vi "measure SEM Measurement.vi"(8 "error in (no error)":errorcluster, 9 "RU":i32, 10 "Center Frequency":dbl, 11 "SA Measurement in":refnum<class "SA Measurement.lvclass">) -> (0 "error out":errorcluster, 2 "Pass?":bool, 3 "SA Measurement out":refnum<class "SA Measurement.lvclass">)   [LabVIEW 2023, in "Spectrum Analyzer.lvlib" / "SA Measurement.lvclass"]
uses:
  SA Measurement.lvclass
  SA Measurement.lvclass/SA Measurement.ctl
  TYPE DEFINITION/Keysight 9020A/TYPE Measurement Preset.ctl
  Spectrum Analyzer.lvlib
  TYPE DEFINITION/TYPE RBW and VBW Select.ctl
  Interface_Spectrum/Interface_Spectrum.lvclass
  TYPE DEFINITION/TYPE Marker Peak Search Type.ctl
  TYPE DEFINITION/TYPE Limit Line Setting Table.ctl
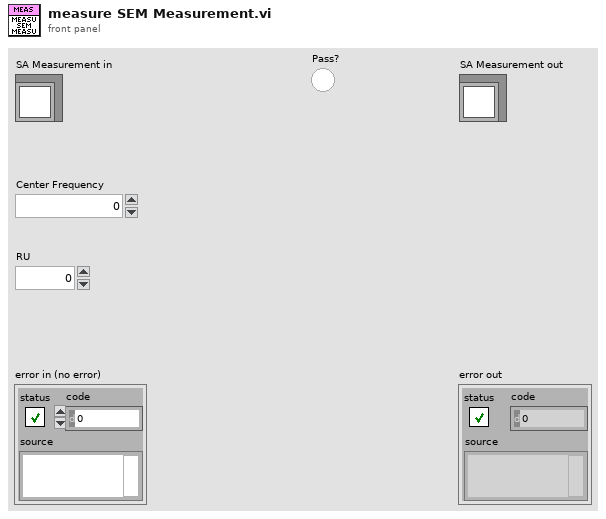
[diagram p1: front panel]
types:
  T1 = typedef "Spectrum Analyzer.lvlib/TYPE Marker Peak Search Type.ctl" = enum16{"Max", "Next Peak"}
  T2 = typedef "Spectrum Analyzer.lvlib/TYPE Limit Line Setting Table.ctl" = cluster{"Limit Line Index":i32, "Frequency Table":dbl[], "Amplitude Table":dbl[], "Name":string}
  T3 = typedef "Spectrum Analyzer.lvlib/TYPE RBW and VBW Select.ctl" = enum16{"Res BW", "Video BW"}
  T4 = typedef "Spectrum Analyzer.lvlib/TYPE Measurement Preset.ctl" = enum16{"Sweep SA Mode", "Channel Power", "Occupied BW", "ACP", "Spurious Emission", "Spurious Emission Mask", "Burst Power (Transmit Power)"}
  T5 = typedef "Spectrum Analyzer.lvlib/TYPE Mask Table for SEM.ctl" = map{enum16{"-10dBm Upper", "-10dBm Lower"}, map{dbl, map{i32, cluster{"Freq":dbl, "Limit":dbl, "dBc Applied?":bool}[]}}}
  T6 = typedef "Spectrum Analyzer.lvlib/TYPE Y-axis Unit.ctl" = enum16{"dBm", "dBmV", "dBuV", "dBpW", "Volt", "Ampere", "Watt"}
  T7 = typedef "Spectrum Analyzer.lvlib/TYPE Reference Level and Atten Param.ctl" = cluster{"Reference Level":dbl, "Atten":i32, "Atten Auto?":bool, "Reference Level Offset":dbl}
  T8 = typedef "Spectrum Analyzer.lvlib/TYPE Start and Stop Frequency.ctl" = cluster{"Start":dbl, "Stop":dbl}
  T9 = typedef "Spectrum Analyzer.lvlib/TYPE Display Trace Mode Select.ctl" = enum16{"Clear Write", "Max Hold", "Min Hold", "Average", "View"}
  T10 = typedef "Spectrum Analyzer.lvlib/TYPE Detect Mode Select.ctl" = enum16{"Det Auto (Normal)", "Auto Peak", "Positive Peak", "Negative Peak", "Sample", "RMS", "Average", "Quasipeak", "CISPR Average", "RMS Average"}
  T11 = cluster{"Trace Mode":T9, "Detector Type":T10, "Detect Auto?":bool}[]
  T12 = typedef "Spectrum Analyzer.lvlib/TYPE Average Mode Select.ctl" = enum16{"Linear(Voltage Avg)", "Video(Log)", "Power"}
  T13 = typedef "Spectrum Analyzer.lvlib/TYPE Marker Value.ctl" = cluster{"X-axis":dbl, "Y-axis":dbl}
  T14 = map{dbl, map{i32, cluster{"Freq":dbl, "Limit":dbl, "dBc Applied?":bool}[]}}
  T15 = map{i32, cluster{"Freq":dbl, "Limit":dbl, "dBc Applied?":bool}[]}
  T16 = cluster{"Freq":dbl, "Limit":dbl, "dBc Applied?":bool}[]
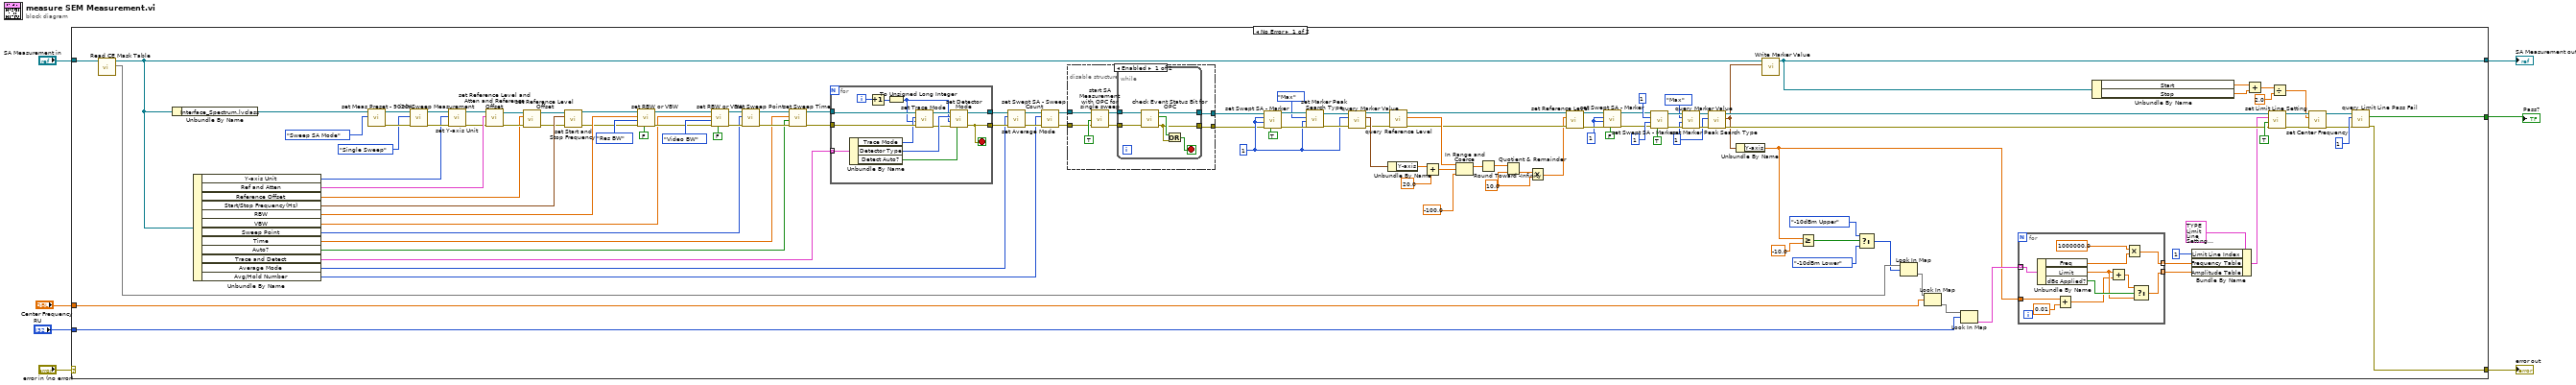
[diagram p0: block diagram]
diagram:
  n1 = case shown="No Error" "error in (no error)" {
    selector: "error in (no error)" -> [_ w167]
    tunnel: [w89 w167] -> w4
    tunnel: [w39 w166] -> w5
    tunnel: "SA Measurement in" -> [w68 w166]
    tunnel: [w88 _] -> w3
    tunnel: "Center Frequency" -> [w66 _]
    tunnel: "RU" -> [w65 _]
    frame No Error {
      w9 = 10.0 ("y")
      w16 = 1 ("Index")
      w31 = 1 ("Index")
      w71 = 1 ("Marker Index")
      n2 = call "Read CE Mask Table.vi"("SA Measurement in"=w68) -> ("Mask Table"=w55:T5, "SA Measurement out"=w41:refnum<class "SA Measurement.lvclass">)  [unwired: 8 in, 1 out]
      n3 = Unbundle By Name(w41) -> ("Interface_Spectrum.lvclass"=w127:refnum<class "Interface_Spectrum.lvclass">)
      n4 = Unbundle By Name(w41) -> ("Y-axis Unit"=w109:T6, "Ref and Atten"=w122:T7, "Reference Offset"=w80:dbl, "Start/Stop Frequency(Hz)"=w92:T8, "RBW"=w121:dbl, "VBW"=w114:dbl, "Sweep Point"=w106:u32, "Time"=w103:dbl, "Auto?"=w102:bool, "Trace and Detect"=w99:T11, "Average Mode"=w96:T12, "Avg/Hold Number"=w93:u32)
      n5 = call-dynamic "set Meas Preset - 9020A.vi"("Measurement Preset"=TYPE_Measurement_Preset."Sweep SA Mode", "Interface_Spectrum in"=w127) -> ("error out"=w124:errorcluster, "Interface_Spectrum out"=w125:refnum<class "Interface_Spectrum.lvclass">)  [unwired: 8 in]
      n6 = call-dynamic "init Sweep Measurement.vi"("error in (no error)"=w124, "Sweep Measurement Mode"=enum16{"Single Sweep", "Continuous Sweep"}."Single Sweep", "Interface_Spectrum in"=w125) -> ("error out"=w112:errorcluster, "Interface_Spectrum out"=w113:refnum<class "Interface_Spectrum.lvclass">)  [unwired: 7 in]
      n7 = call-dynamic "set Y-axis Unit.vi"("error in (no error)"=w112, "Y-axis Unit"=w109, "Interface_Spectrum in"=w113) -> ("error out"=w110:errorcluster, "Interface_Spectrum out"=w111:refnum<class "Interface_Spectrum.lvclass">)  [unwired: 7 in]
      n8 = call-dynamic "set Reference Level and Atten and Reference Offset.vi"("error in (no error)"=w110, "Reference Level, Atten, Reference Offset"=w122, "Interface_Spectrum in"=w111) -> ("error out"=w83:errorcluster, "Interface_Spectrum out"=w84:refnum<class "Interface_Spectrum.lvclass">)  [unwired: 7 in]
      n9 = call-dynamic "set Reference Level Offset.vi"("error in (no error)"=w83, "Reference Level Offset"=w80, "Interface_Spectrum in"=w84) -> ("error out"=w81:errorcluster, "Interface_Spectrum out"=w82:refnum<class "Interface_Spectrum.lvclass">)  [unwired: 7 in]
      n10 = call-dynamic "set Start and Stop Frequency.vi"("error in (no error)"=w81, "Start/Stop Frequency(Hz)"=w92, "Interface_Spectrum in"=w82) -> ("error out"=w90:errorcluster, "Interface_Spectrum out"=w91:refnum<class "Interface_Spectrum.lvclass">)  [unwired: 7 in]
      n11 = call-dynamic "set RBW or VBW.vi"("BW Auto?"=FALSE, "error in (no error)"=w90, "BW Type"=TYPE_RBW_and_VBW_Select."Res BW", "BW Value (Hz)"=w121, "Interface_Spectrum in"=w91) -> ("error out"=w115:errorcluster, "Interface_Spectrum out"=w116:refnum<class "Interface_Spectrum.lvclass">)  [unwired: 5 in]
      n12 = call-dynamic "set RBW or VBW.vi"("BW Auto?"=FALSE, "error in (no error)"=w115, "BW Type"=TYPE_RBW_and_VBW_Select."Video BW", "BW Value (Hz)"=w114, "Interface_Spectrum in"=w116) -> ("error out"=w107:errorcluster, "Interface_Spectrum out"=w108:refnum<class "Interface_Spectrum.lvclass">)  [unwired: 5 in]
      n13 = call-dynamic "set Sweep Point.vi"("error in (no error)"=w107, "Sweep Point"=w106, "Interface_Spectrum in"=w108) -> ("error out"=w104:errorcluster, "Interface_Spectrum out"=w105:refnum<class "Interface_Spectrum.lvclass">)  [unwired: 7 in]
      n14 = call-dynamic "set Sweep Time.vi"("error in (no error)"=w104, "Sweep Time Auto?"=w102, "Sweep Time(sec)"=w103, "Interface_Spectrum in"=w105) -> ("error out"=w100:errorcluster, "Interface_Spectrum out"=w101:refnum<class "Interface_Spectrum.lvclass">)  [unwired: 6 in]
      n15 = for {
        tunnel: w101 -> [w164]
        tunnel: w100 -> [w163]
        tunnel: w99 -> [w165] mode=indexing
        tunnel: [w153] -> w97
        tunnel: [w154] -> w98
        i -> [w162]
        stop <- w153 stop-if-true
        n16 = Unbundle By Name(w165) -> ("Trace Mode"=w160:T9, "Detector Type"=w158:T10, "Detect Auto?"=w155:bool)
        n17 = Increment(x=w162) -> (x+1=w161:i32)
        n18 = To Unsigned Long Integer(number=w161) -> (unsigned 32bit integer=w156:u32)
        n19 = call-dynamic "set Trace Mode.vi"("error in (no error)"=w163, "Trace Index"=w156, "Trace Mode"=w160, "Interface_Spectrum in"=w164) -> ("error out"=w157:errorcluster, "Interface_Spectrum out"=w159:refnum<class "Interface_Spectrum.lvclass">)  [unwired: 6 in]
        n20 = call-dynamic "set Detector Mode.vi"("Detect Auto?"=w155, "error in (no error)"=w157, "Trace Index"=w156, "Detector Type"=w158, "Interface_Spectrum in"=w159) -> ("error out"=w153:errorcluster, "Interface_Spectrum out"=w154:refnum<class "Interface_Spectrum.lvclass">)  [unwired: 5 in]
      }
      n21 = call-dynamic "set Average Mode.vi"("error in (no error)"=w97, "Average Mode"=w96, "Interface_Spectrum in"=w98) -> ("error out"=w94:errorcluster, "Interface_Spectrum out"=w95:refnum<class "Interface_Spectrum.lvclass">)  [unwired: 7 in]
      n22 = call-dynamic "set Swept SA - Sweep Count.vi"("error in (no error)"=w94, "Sweep Count"=w93, "Interface_Spectrum in"=w95) -> ("error out"=w85:errorcluster, "Interface_Spectrum out"=w86:refnum<class "Interface_Spectrum.lvclass">)  [unwired: 7 in]
      n23 = disable-structure shown="Enabled" {
        disable-tunnel: [w142 w152] -> w15
        disable-tunnel: [w141 _] -> w14
        disable-tunnel: w86 -> [w140 w152]
        disable-tunnel: w85 -> [w139 _]
        frame Enabled {
          n24 = call-dynamic "start SA Measurement with OPC for single sweep.vi"("error in (no error)"=w139, "with OPC?"=TRUE, "Interface_Spectrum in"=w140) -> ("error out"=w143:errorcluster, "Interface_Spectrum out"=w144:refnum<class "Interface_Spectrum.lvclass">)  [unwired: 7 in]
          n25 = while {
            tunnel: w144 -> [w151]
            tunnel: w143 -> [w150]
            tunnel: [w147] -> w141
            tunnel: [w146] -> w142
            stop <- w148 stop-if-true
            n26 = call-dynamic "check Event Status Bit for OPC.vi"("error in (no error)"=w150, "Interface_Spectrum in"=w151) -> ("error out"=w147:errorcluster, "OPC Bit Changed?"=w149:bool, "Interface_Spectrum out"=w146:refnum<class "Interface_Spectrum.lvclass">)  [unwired: 7 in]
            n27 = Or(x=w149, y=w147) -> (x .or. y?=w148:bool)
          }
        }
        frame Disabled {
        }
      }
      n28 = call-dynamic "set Swept SA - Marker.vi"("On?"=TRUE, "error in (no error)"=w14, "trace"=w31, "Index"=w31, "Interface_Spectrum in"=w15) -> ("error out"=w35:errorcluster, "Interface_Spectrum out"=w36:refnum<class "Interface_Spectrum.lvclass">)  [unwired: 5 in]
      n29 = call-dynamic "set Marker Peak Search Type.vi"("error in (no error)"=w35, "Marker Index"=w31, "Peak Search Type"=TYPE_Marker_Peak_Search_Type."Max", "Interface_Spectrum in"=w36) -> ("error out"=w32:errorcluster, "Interface_Spectrum out"=w33:refnum<class "Interface_Spectrum.lvclass">)  [unwired: 6 in]
      n30 = call-dynamic "query Marker Value.vi"("error in (no error)"=w32, "Marker Index"=w31, "Interface_Spectrum in"=w33) -> ("error out"=w26:errorcluster, "Marker Value"=w28:T13, "Interface_Spectrum out"=w27:refnum<class "Interface_Spectrum.lvclass">)  [unwired: 6 in]
      n31 = Unbundle By Name(w28) -> ("Y-axis"=w30:dbl)
      n32 = call-dynamic "query Reference Level.vi"("error in (no error)"=w26, "Interface_Spectrum in"=w27) -> ("error out"=w21:errorcluster, "Ref Level"=w24:dbl, "Interface_Spectrum out"=w25:refnum<class "Interface_Spectrum.lvclass">)  [unwired: 7 in]
      n33 = Add(x=w30, y=20.0) -> (x+y=w23:dbl)
      n34 = In Range and Coerce(upper limit=w24, x=w23, lower limit=-100.0) -> (coerced(x)=w20:dbl)  [unwired: 1 out]
      n35 = Round Toward -Infinity(1:w20) -> (0:w11:dbl)
      n36 = Quotient & Remainder(x=w11, y=w9) -> (floor(x/y)=w10:dbl)  [unwired: 1 out]
      n37 = Multiply(x=w10, y=w9) -> (x*y=w8:dbl)
      n38 = call-dynamic "set Reference Level.vi"("error in (no error)"=w21, "Reference Level"=w8, "Interface_Spectrum in"=w25) -> ("error out"=w18:errorcluster, "Interface_Spectrum out"=w19:refnum<class "Interface_Spectrum.lvclass">)  [unwired: 7 in]
      n39 = call-dynamic "set Swept SA - Marker.vi"("On?"=FALSE, "error in (no error)"=w18, "trace"=w16, "Index"=w16, "Interface_Spectrum in"=w19) -> ("error out"=w12:errorcluster, "Interface_Spectrum out"=w13:refnum<class "Interface_Spectrum.lvclass">)  [unwired: 5 in]
      n40 = call-dynamic "set Swept SA - Marker.vi"("On?"=TRUE, "error in (no error)"=w12, "trace"=1, "Index"=1, "Interface_Spectrum in"=w13) -> ("error out"=w75:errorcluster, "Interface_Spectrum out"=w76:refnum<class "Interface_Spectrum.lvclass">)  [unwired: 5 in]
      n41 = call-dynamic "set Marker Peak Search Type.vi"("error in (no error)"=w75, "Marker Index"=w71, "Peak Search Type"=TYPE_Marker_Peak_Search_Type."Max", "Interface_Spectrum in"=w76) -> ("error out"=w72:errorcluster, "Interface_Spectrum out"=w73:refnum<class "Interface_Spectrum.lvclass">)  [unwired: 6 in]
      n42 = call-dynamic "query Marker Value.vi"("error in (no error)"=w72, "Marker Index"=w71, "Interface_Spectrum in"=w73) -> ("error out"=w69:errorcluster, "Marker Value"=w40:T13, "Interface_Spectrum out"=w70:refnum<class "Interface_Spectrum.lvclass">)  [unwired: 6 in]
      n43 = Unbundle By Name(w40) -> ("Y-axis"=w58:dbl)
      n44 = call "Write Marker Value.vi"("Marker Value"=w40, "SA Measurement in"=w41) -> ("SA Measurement out"=w39:refnum<class "SA Measurement.lvclass">)  [unwired: 8 in, 1 out]
      n45 = Greater Or Equal?(x=w58, y=-10.0) -> (x >= y?=w56:bool)
      n46 = Select(t=enum16{"-10dBm Upper", "-10dBm Lower"}."-10dBm Upper" ("key"), s=w56, f=enum16{"-10dBm Upper", "-10dBm Lower"}."-10dBm Lower" ("key")) -> (s? t:f=w52:enum16{"-10dBm Upper", "-10dBm Lower"})
      n47 = Look In Map(map=w55, key=w52) -> (value=w51:T14)  [unwired: 1 in, 1 out]
      n48 = Look In Map(map=w51, key=w66) -> (value=w67:T15)  [unwired: 1 in, 1 out]
      n49 = Look In Map(map=w67, key=w65) -> (value=w64:T16)  [unwired: 1 in, 1 out]
      n50 = for {
        tunnel: w64 -> [w138] mode=indexing
        tunnel: [w135] -> w61 mode=indexing
        tunnel: [w133] -> w60 mode=indexing
        tunnel: w58 -> [w130]
        n51 = Unbundle By Name(w138) -> ("Freq"=w137:dbl, "Limit"=w131:dbl, "dBc Applied?"=w134:bool)
        n52 = Add(x=w130, y=0.01) -> (x+y=w129:dbl)
        n53 = Add(x=w131, y=w129) -> (x+y=w132:dbl)
        n54 = Multiply(x=1000000.0, y=w137) -> (x*y=w135:dbl)
        n55 = Select(t=w132, s=w134, f=w131) -> (s? t:f=w133:dbl)
      }
      n56 = Unbundle By Name(w39) -> ("Start"=w46:dbl, "Stop"=w45:dbl)
      n57 = Bundle By Name(cluster=T2 {"Limit Line Index"=1, "Frequency Table"=[1000000000.0, 2000000000.0, 3000000000.0], "Amplitude Table"=[-60.0, -50.0, -40.0], "Name"=""} ("Limit Line Setting"), "Limit Line Index"=1, "Frequency Table"=w61, "Amplitude Table"=w60) -> (w38:T2)
      n58 = Add(x=w46, y=w45) -> (x+y=w44:dbl)
      n59 = call-dynamic "set Limit Line Setting.vi"("error in (no error)"=w69, "Turn On?"=TRUE, "Limit Line Setting"=w38, "Interface_Spectrum in"=w70) -> ("error out"=w49:errorcluster, "Interface_Spectrum out"=w50:refnum<class "Interface_Spectrum.lvclass">)  [unwired: 6 in]
      n60 = Divide(x=w44, y=2.0) -> (x/y=w42:dbl)
      n61 = call-dynamic "set Center Frequency.vi"("error in (no error)"=w49, "Center Frequency (Hz)"=w42, "Interface_Spectrum in"=w50) -> ("error out"=w47:errorcluster, "Interface_Spectrum out"=w48:refnum<class "Interface_Spectrum.lvclass">)  [unwired: 7 in]
      n62 = call-dynamic "query Limit Line Pass Fail.vi"("error in (no error)"=w47, "Limit Line Index"=1, "Interface_Spectrum in"=w48) -> ("error out"=w89:errorcluster, "Pass?"=w88:bool)  [unwired: 6 in, 1 out]
    }
    frame Error {
    }
  }
  "error out" <- w4
  "SA Measurement out" <- w5
  "Pass?" <- w3
